vi "Low-Level HTTP Request AWS v4.vi"(5 "Request Options":T2={"request headers"=[], "request parameters"=[], "request body"="", "region handling"=enum."use region everywhere", "URL formatting"=enum."region."}, 7 "HTTP-Verb":string(combo)="GET", 8 "error in (no error)":errorcluster, 9 "URL Suffix":string, 10 "URL Prefix":string, 11 "AWS Core in":refnum<class "HTTP Request.lvclass">) -> (0 "error out":errorcluster, 1 "Response":T1, 2 "Call Result":string, 3 "AWS Core out":refnum<class "HTTP Request.lvclass">)   [LabVIEW 2015, in "NI_AWS_Core.lvlib" / "HTTP Request.lvclass"]
doc: "This core implementation of AWS v4 HTTP requests may be used to implement special requests or API calls not present in this toolkit."
uses:
  HTTP Request.lvclass
  Request Options.ctl
  Name Value Pair.ctl
  Region handling.ctl
  URL formatting.ctl
  Response.ctl
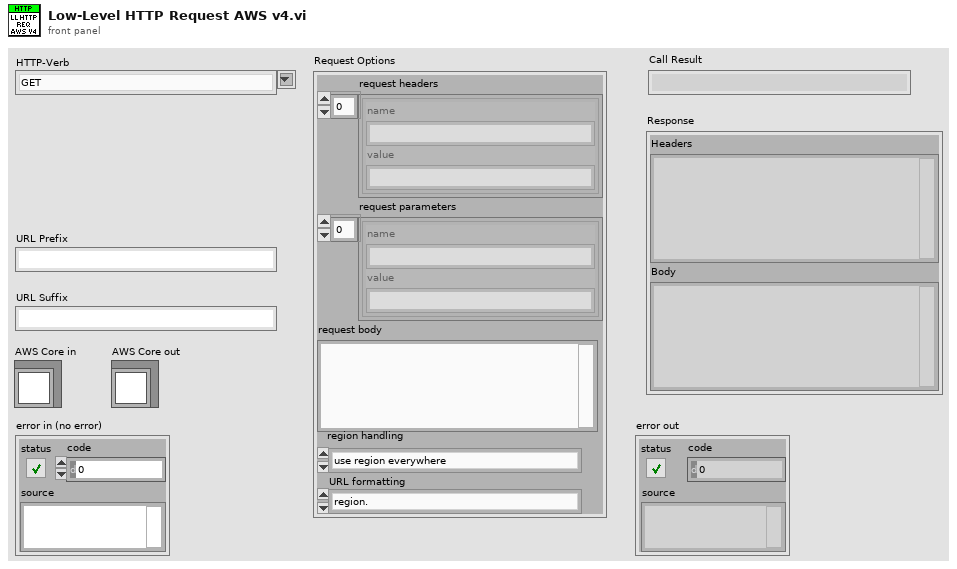
[diagram p1: front panel]
types:
  T1 = typedef "NI_AWS_Core.lvlib/HTTP Request.lvclass/Response.ctl" = cluster{"Headers":string, "Body":string}
  T2 = typedef "NI_AWS_Core.lvlib/HTTP Request.lvclass/Request Options.ctl" = cluster{"request headers":T3[], "request parameters":T3[], "request body":string, "region handling":T4, "URL formatting":T5}
  T3 = typedef "NI_AWS_Core.lvlib/HTTP Request.lvclass/Name Value Pair.ctl" = cluster{"name":string, "value":string}
  T4 = typedef "NI_AWS_Core.lvlib/HTTP Request.lvclass/Region handling.ctl" = enum16{"use region everywhere", "use region (authentication only)", "use region (URL only)", "ignore region everwhere"}
  T5 = typedef "NI_AWS_Core.lvlib/HTTP Request.lvclass/URL formatting.ctl" = enum16{"region-", "region."}
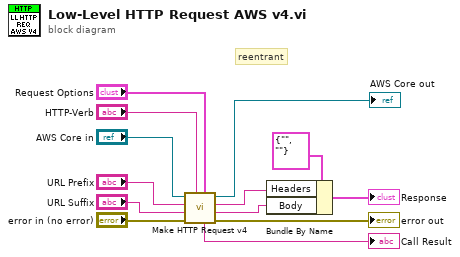
[diagram p0: block diagram]
diagram:
  # "reentrant"
  n1 = call "Make HTTP Request v4.vi"("Request Options"="Request Options", "HTTP-Verb"="HTTP-Verb", "error in"="error in (no error)", "URL Suffix"="URL Suffix", "URL Prefix"="URL Prefix", "AWS Core in"="AWS Core in") -> ("error out"=→"error out":errorcluster, "response body"=w3:string, "response headers"=w2:string, "AWS Core out"=→"AWS Core out":refnum<class "HTTP Request.lvclass">, "Call Result"=→"Call Result":string)  [unwired: 1 in]
  n2 = Bundle By Name(cluster=T1 {"Headers"="", "Body"=""} ("Response"), "Headers"=w2, "Body"=w3) -> (→"Response":T1)
